vi "Init.vi"(8 "error in (no error)":errorcluster, 11 "Data in":refnum<class "CTI_Bus.lvclass">) -> (0 "error out":errorcluster, 3 "Data out":refnum<class "CTI_Bus.lvclass">)   [LabVIEW 2021, in "CTI_Bus.lvclass"]
doc: "Abstract Data Classes 2.1.1.12\nTim Streeter - TSA\nCopyright (c) 2024, TSAOmni-Bus 2.0.1.6\nTim - TSA\nCopyright (c) 2024, TSA"
uses:
  CTI_Bus.lvclass
  C:/Program Files (x86)/National Instruments/LabVIEW 2021/vi.lib/TSA/Omni-Bus/Omni-Bus/Bus Access/Bus_Access.lvclass
  CTI_Bus.lvclass/CTI_Bus.ctl
  Channels/CTI_Channel.lvclass
  <vilib>/TSA/Abstract Data Classes/Abs_Types/Type/Abs_Type.lvclass
  <vilib>/TSA/Omni-Bus/Omni-Bus/Bus Access/Bus_Access.lvclass/Bus_Access.ctl
  <vilib>/TSA/Omni-Bus/Omni-Bus/Bus Access/Properties/Write Values.vi
  <vilib>/TSA/Omni-Bus/Omni-Bus/Bus Access/Properties/Write Tags.vi
  Properties/Read Session.vi
  <vilib>/CTI/CTI Drivers/CTI/Session/Session.lvclass
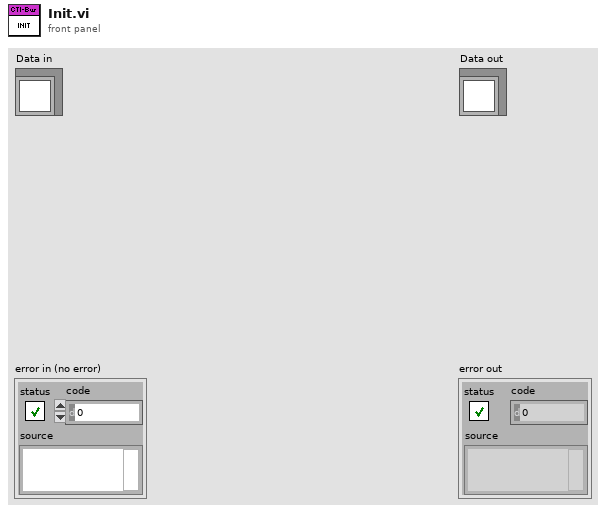
[diagram p1: front panel]
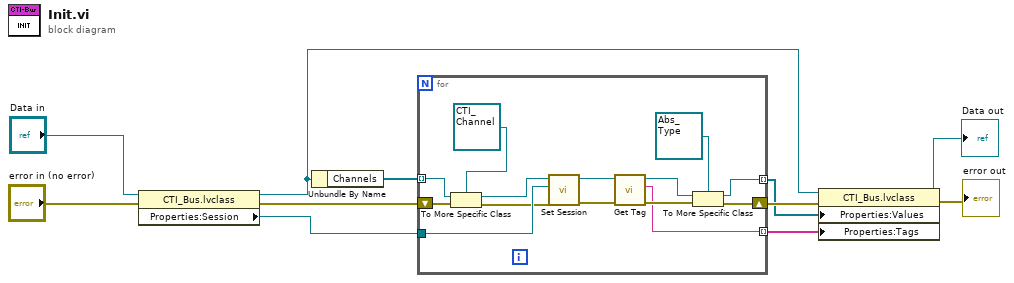
[diagram p0: block diagram]
diagram:
  n1 = property class="CTI_Bus.lvclass"(reference="Data in", error in="error in (no error)") -> (reference out=w4:refnum<class "CTI_Bus.lvclass">, error out=w3:errorcluster, "Properties:Session"=w2:refnum<class "Session.lvclass">)
  n2 = Unbundle By Name(w4) -> ("Channels"=w11:refnum<class "Abs_Type.lvclass">[])
  n3 = for {
    tunnel: w11 -> [w15] mode=indexing
    shift-right: [w24] -> w10
    shift-left: w3 -> [w16]
    tunnel: [w25] -> w9 mode=indexing
    tunnel: w2 -> [w22]
    tunnel: [w17] -> w1 mode=indexing
    n4 = To More Specific Class(target class=refnum<class "CTI_Channel.lvclass"> refnum ("CTI_Channel in"), reference=w15, error in=w16) -> (specific class reference=w13:refnum<class "CTI_Channel.lvclass">, error out=w12:errorcluster)
    n5 = call-dynamic "Set Session.vi"("error in (no error)"=w12, "Session"=w22, "CTI_Channel in"=w13) -> ("error out"=w21:errorcluster, "CTI_Channel out"=w20:refnum<class "CTI_Channel.lvclass">)  [unwired: 7 in]
    n6 = call-dynamic "Get Tag.vi"("error in (no error)"=w21, "CTI_Channel in"=w20) -> ("error out"=w18:errorcluster, "Tag"=w17:string, "CTI_Channel out"=w19:refnum<class "CTI_Channel.lvclass">)  [unwired: 7 in]
    n7 = To More Specific Class(target class=refnum<class "Abs_Type.lvclass"> refnum ("Data in"), reference=w19, error in=w18) -> (specific class reference=w25:refnum<class "Abs_Type.lvclass">, error out=w24:errorcluster)
  }
  n8 = property class="CTI_Bus.lvclass"(reference=w4, error in=w10, "Properties:Values"=w9, "Properties:Tags"=w1) -> (reference out=→"Data out":refnum<class "CTI_Bus.lvclass">, error out=→"error out":errorcluster)
